vi "Motor_Open.vi"() -> ()   [LabVIEW 2016]
uses:
  <vilib>/Rock Robotics/WPI/SafetyOutput/WPI_SafetyOutputConfigMenu.ctl
  <vilib>/Rock Robotics/WPI/ThirdParty/CanMotor/TalonSRX/WPI_CANTalonSRX_APIControlMode.ctl
  ArgosLib/Drive/MotorControl/TypeDefs/RobotDriveMotorSelectorEnum.ctl
  <vilib>/Rock Robotics/WPI/ThirdParty/CanMotor/TalonSRX/WPI_CANTalonSRX_APIFeedbackSelect.ctl
  Global_Var-RefNum/Global_Var_Drive.vi
  ArgosLib/Drive/MotorControl/RobotDriveOpen6MotorWithTalonSRX.vi
  ArgosLib/ArgosLib.lvlib
panel:
  in  "Left Motor 1 Inverted_P":bool
  in  "Left Motor 2 Inverted_P":bool
  in  "Right Motor 1 Inverted_P":bool
  in  "Right Motor 2 Inverted_P":bool
  in  "Left Motor 1 Inverted":bool
  in  "Left Motor 2 Inverted":bool
  in  "Right Motor 1 Inverted":bool
  in  "Right Motor 2 Inverted":bool
  # "Practice"
  # "Competition"
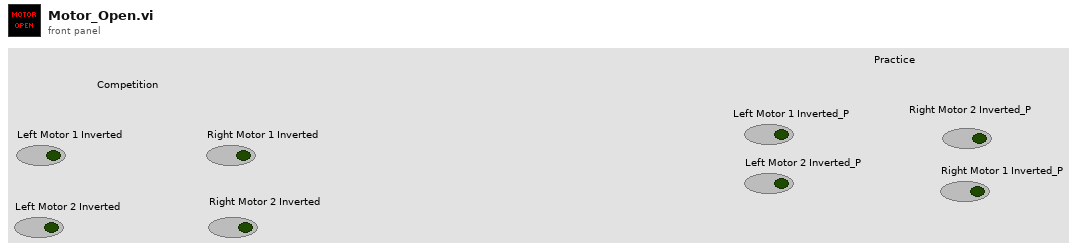
[diagram p1: front panel]
types:
  T1 = typedef "WPI_SafetyOutputConfigMenu.ctl" = enum16{"Enable", "Disable"}
  T2 = typedef "WPI_CANTalonSRX_APIControlMode.ctl" = enum8{"Percent VBus", "Speed", "Position", "Slave", "Unchanged / Invalid", "Voltage Compensation", "Current", "Motion Profile", "Motion Magic"}
  T3 = typedef "ArgosLib.lvlib/RobotDriveMotorSelectorEnum.ctl" = enum16{"Left Motor 1", "Right Motor 1", "Left Motor 2", "Right Motor 2", "Left Motor 3", "Right Motor 3"}
  T4 = typedef "WPI_RobotDriveDevRef.ctl" = cluster{"DevStatus":errorcluster, "Motors[]":T5[], "Square Inputs":bool, "Max Output":dbl}
  T5 = typedef "WPI_MotorControlDeviceRef.ctl" = cluster{"DeviceStatus":errorcluster, "Type":T6, "PWM":cluster{"PWM Channel":T7, "DeadBand":T8}, "CAN":cluster{"Device Number":u8, "SetOutput VI Ref":variant, "GetOutput VI Ref":variant, "Enable VI Ref":variant, "Disable VI Ref":variant, "Data":variant}, "Invert":bool}
  T6 = typedef "WPI_MotorControlType.ctl" = enum16{"PWM", "CAN"}
  T7 = typedef "FPGA_DIOPWMChannel.ctl" = enum8{"PWM 0", "PWM 1", "PWM 2", "PWM 3", "PWM 4", "PWM 5", "PWM 6", "PWM 7", "PWM 8", "PWM 9", "PWM MXP 0", "PWM MXP 1", "PWM MXP 2", "PWM MXP 3", "PWM MXP 4", "PWM MXP 5", "PWM MXP 6", "PWM MXP 7", "PWM MXP 8", "PWM MXP 9", "Invalid"}
  T8 = typedef "WPI_PWMDeadband.ctl" = cluster{"Name":string, "maxPositivePwm":i32, "minPositivePwm":i32, "centerPwm":i32, "maxNegativePwm":i32, "minNegativePwm":i32, "angularRange":u16}
  T9 = typedef "WPI_CANTalonSRX_APIFeedbackSelect.ctl" = enum16{"Digital Quadrature Encoder", "Analog Potentiometer", "Analog Encoder", "Count on Quad-A (Rising-Edge)", "Count on Quad-A (Falling-Edge)", "CTR Magnetic Enc (Absolute)", "CTR Magnetic Enc (Relative)", "Pulse Width"}
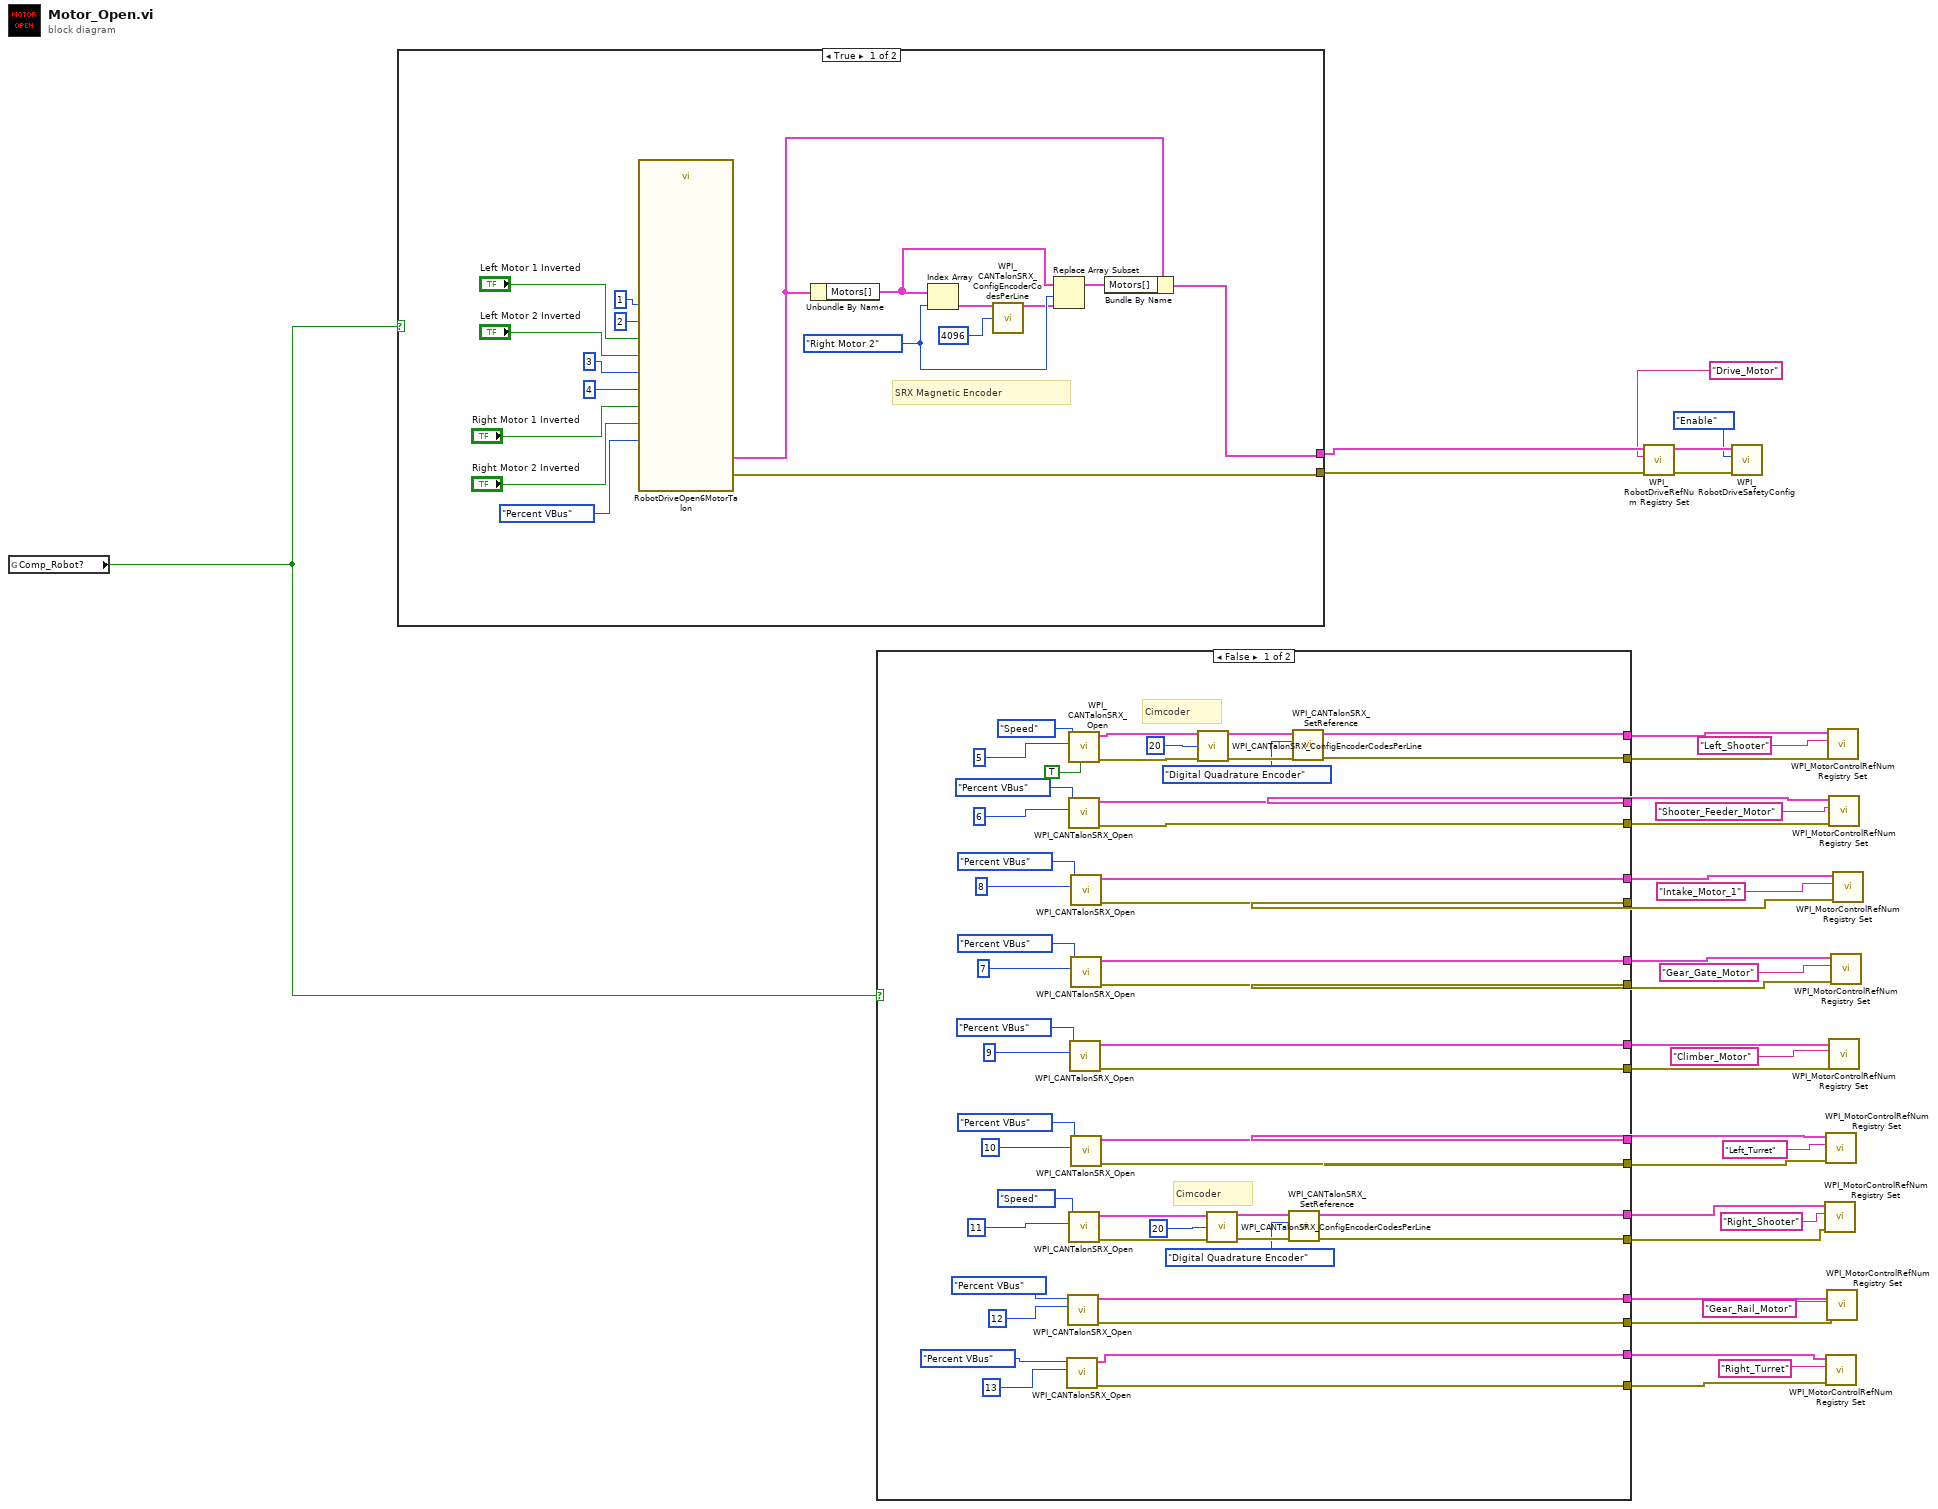
[diagram p0: block diagram]
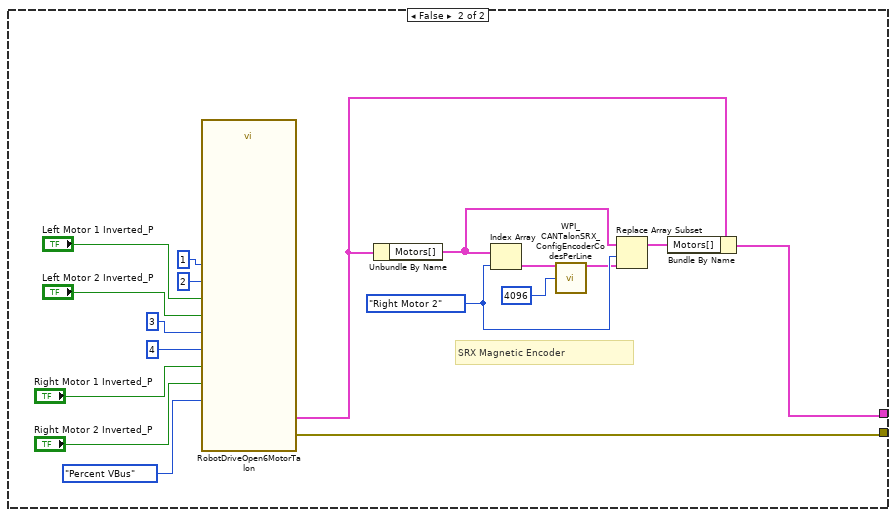
[diagram p2: hidden frame]
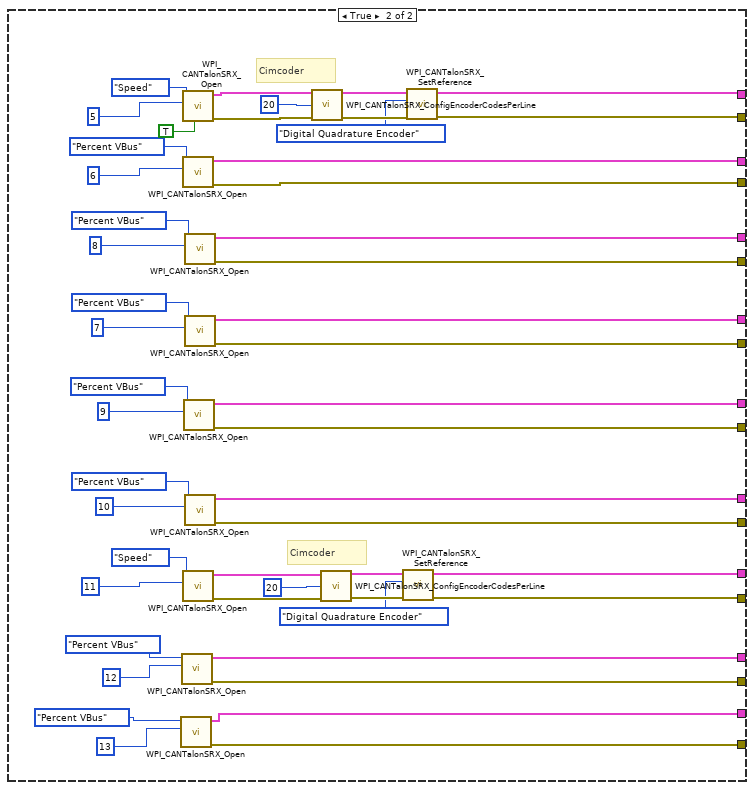
[diagram p3: hidden frame]
diagram:
  n1 = global read "Global_Var_Drive.vi" "Comp_Robot?"() -> (w4:bool)
  n2 = case shown="True" w4 {
    tunnel: [w43 w61] -> w34
    tunnel: [w35 w53] -> w33
    frame True {
      w39 = RobotDriveMotorSelectorEnum."Right Motor 2" ("Motor Selector Enum")
      # "SRX Magnetic Encoder"
      n3 = call-poly "RobotDriveOpen6MotorTalon.vi"("Left Motor 1"=u8 1, "Left Motor 2"=u8 2, "Right Motor 1"=u8 3, "Right Motor 2"=u8 4, "Left Motor 1 Inverted"="Left Motor 1 Inverted", "Right Motor 1 Inverted"="Right Motor 1 Inverted", "Left Motor 2 Inverted"="Left Motor 2 Inverted", "Right Motor 2 Inverted"="Right Motor 2 Inverted", "Control Mode"=WPI_CANTalonSRX_APIControlMode."Percent VBus") -> ("RobotDriveDevRef"=w36:T4, "error out"=w43:errorcluster)  [unwired: 17 in]
      n4 = Unbundle By Name(w36) -> ("Motors[]"=w40:T5[])
      n5 = Index Array(array=w40, index=w39) -> (element=w42:T5)
      n6 = call <vilib>:"WPI_CANTalonSRX_ConfigEncoderCodesPerLine.vi"("CAN Talon SRX Ref"=w42, "Number Encoder Lines\n(Counts Per Rotation)"=u32 4096 ("Number Encoder Lines\n(Counts Per Rotation)")) -> ("CAN Talon SRX Ref"=w38:T5)  [unwired: 12 in, 1 out]
      n7 = Replace Array Subset(array=w40, new element=w38, index=w39) -> (w37:T5[])
      n8 = Bundle By Name(cluster=w36, "Motors[]"=w37) -> (w35:T4)
    }
    frame False {
      w57 = RobotDriveMotorSelectorEnum."Right Motor 2" ("Motor Selector Enum")
      # "SRX Magnetic Encoder"
      n9 = call-poly "RobotDriveOpen6MotorTalon.vi"("Left Motor 1"=u8 1, "Left Motor 2"=u8 2, "Right Motor 1"=u8 3, "Right Motor 2"=u8 4, "Left Motor 1 Inverted"="Left Motor 1 Inverted_P", "Right Motor 1 Inverted"="Right Motor 1 Inverted_P", "Left Motor 2 Inverted"="Left Motor 2 Inverted_P", "Right Motor 2 Inverted"="Right Motor 2 Inverted_P", "Control Mode"=WPI_CANTalonSRX_APIControlMode."Percent VBus") -> ("RobotDriveDevRef"=w54:T4, "error out"=w61:errorcluster)  [unwired: 17 in]
      n10 = Unbundle By Name(w54) -> ("Motors[]"=w58:T5[])
      n11 = Index Array(array=w58, index=w57) -> (element=w60:T5)
      n12 = call <vilib>:"WPI_CANTalonSRX_ConfigEncoderCodesPerLine.vi"("CAN Talon SRX Ref"=w60, "Number Encoder Lines\n(Counts Per Rotation)"=u32 4096 ("Number Encoder Lines\n(Counts Per Rotation)")) -> ("CAN Talon SRX Ref"=w56:T5)  [unwired: 12 in, 1 out]
      n13 = Replace Array Subset(array=w58, new element=w56, index=w57) -> (w55:T5[])
      n14 = Bundle By Name(cluster=w54, "Motors[]"=w55) -> (w53:T4)
    }
  }
  n15 = case shown="False" w4 {
    tunnel: [w75 w124] -> w22
    tunnel: [w73 w122] -> w21
    tunnel: [w93 w142] -> w20
    tunnel: [w107 w156] -> w19
    tunnel: [w94 w143] -> w18
    tunnel: [w106 w155] -> w17
    tunnel: [w88 w137] -> w16
    tunnel: [w105 w154] -> w15
    tunnel: [w92 w141] -> w14
    tunnel: [w104 w153] -> w13
    tunnel: [w91 w140] -> w12
    tunnel: [w103 w152] -> w11
    tunnel: [w79 w128] -> w10
    tunnel: [w77 w126] -> w9
    tunnel: [w90 w139] -> w7
    tunnel: [w98 w147] -> w6
    tunnel: [w97 w146] -> w3
    tunnel: [w89 w138] -> w1
    frame False {
      # "Cimcoder"
      # "Cimcoder"
      n16 = call <vilib>:"WPI_CANTalonSRX_Open.vi"("Device Number"=u8 13, "Control Mode"=WPI_CANTalonSRX_APIControlMode."Percent VBus") -> ("error out"=w97:errorcluster, "CAN Talon SRX Ref"=w89:T5)  [unwired: 8 in]
      n17 = call <vilib>:"WPI_CANTalonSRX_Open.vi"("Device Number"=u8 12, "Control Mode"=WPI_CANTalonSRX_APIControlMode."Percent VBus") -> ("error out"=w98:errorcluster, "CAN Talon SRX Ref"=w90:T5)  [unwired: 8 in]
      n18 = call <vilib>:"WPI_CANTalonSRX_Open.vi"("Invert"=TRUE, "Device Number"=u8 5, "Control Mode"=WPI_CANTalonSRX_APIControlMode."Speed") -> ("error out"=w81:errorcluster, "CAN Talon SRX Ref"=w87:T5)  [unwired: 7 in]
      n19 = call <vilib>:"WPI_CANTalonSRX_Open.vi"("Device Number"=u8 6, "Control Mode"=WPI_CANTalonSRX_APIControlMode."Percent VBus") -> ("error out"=w107:errorcluster, "CAN Talon SRX Ref"=w93:T5)  [unwired: 8 in]
      n20 = call <vilib>:"WPI_CANTalonSRX_Open.vi"("Device Number"=u8 11, "Control Mode"=WPI_CANTalonSRX_APIControlMode."Speed") -> ("error out"=w80:errorcluster, "CAN Talon SRX Ref"=w84:T5)  [unwired: 8 in]
      n21 = call <vilib>:"WPI_CANTalonSRX_Open.vi"("Device Number"=u8 9, "Control Mode"=WPI_CANTalonSRX_APIControlMode."Percent VBus") -> ("error out"=w104:errorcluster, "CAN Talon SRX Ref"=w92:T5)  [unwired: 8 in]
      n22 = call <vilib>:"WPI_CANTalonSRX_Open.vi"("Device Number"=u8 8, "Control Mode"=WPI_CANTalonSRX_APIControlMode."Percent VBus") -> ("error out"=w106:errorcluster, "CAN Talon SRX Ref"=w94:T5)  [unwired: 8 in]
      n23 = call <vilib>:"WPI_CANTalonSRX_Open.vi"("Device Number"=u8 7, "Control Mode"=WPI_CANTalonSRX_APIControlMode."Percent VBus") -> ("error out"=w105:errorcluster, "CAN Talon SRX Ref"=w88:T5)  [unwired: 8 in]
      n24 = call <vilib>:"WPI_CANTalonSRX_Open.vi"("Device Number"=u8 10, "Control Mode"=WPI_CANTalonSRX_APIControlMode."Percent VBus") -> ("error out"=w103:errorcluster, "CAN Talon SRX Ref"=w91:T5)  [unwired: 8 in]
      n25 = call <vilib>:"WPI_CANTalonSRX_ConfigEncoderCodesPerLine.vi"("CAN Talon SRX Ref"=w87, "Number Encoder Lines\n(Counts Per Rotation)"=u32 20 ("Number Encoder Lines\n(Counts Per Rotation)"), "error in (no error)"=w81) -> ("CAN Talon SRX Ref"=w86:T5, "error out"=w74:errorcluster)  [unwired: 11 in]
      n26 = call <vilib>:"WPI_CANTalonSRX_ConfigEncoderCodesPerLine.vi"("CAN Talon SRX Ref"=w84, "Number Encoder Lines\n(Counts Per Rotation)"=u32 20 ("Number Encoder Lines\n(Counts Per Rotation)"), "error in (no error)"=w80) -> ("CAN Talon SRX Ref"=w83:T5, "error out"=w78:errorcluster)  [unwired: 11 in]
      n27 = call <vilib>:"WPI_CANTalonSRX_SetReference.vi"("error in (no error)"=w78, "Feedback Reference"=WPI_CANTalonSRX_APIFeedbackSelect."Digital Quadrature Encoder", "CAN Talon SRX Ref"=w83) -> ("error out"=w77:errorcluster, "CAN Talon SRX Ref"=w79:T5)  [unwired: 7 in]
      n28 = call <vilib>:"WPI_CANTalonSRX_SetReference.vi"("error in (no error)"=w74, "Feedback Reference"=WPI_CANTalonSRX_APIFeedbackSelect."Digital Quadrature Encoder", "CAN Talon SRX Ref"=w86) -> ("error out"=w73:errorcluster, "CAN Talon SRX Ref"=w75:T5)  [unwired: 7 in]
    }
    frame True {
      # "Cimcoder"
      # "Cimcoder"
      n29 = call <vilib>:"WPI_CANTalonSRX_Open.vi"("Device Number"=u8 13, "Control Mode"=WPI_CANTalonSRX_APIControlMode."Percent VBus") -> ("error out"=w146:errorcluster, "CAN Talon SRX Ref"=w138:T5)  [unwired: 8 in]
      n30 = call <vilib>:"WPI_CANTalonSRX_Open.vi"("Device Number"=u8 12, "Control Mode"=WPI_CANTalonSRX_APIControlMode."Percent VBus") -> ("error out"=w147:errorcluster, "CAN Talon SRX Ref"=w139:T5)  [unwired: 8 in]
      n31 = call <vilib>:"WPI_CANTalonSRX_Open.vi"("Invert"=TRUE, "Device Number"=u8 5, "Control Mode"=WPI_CANTalonSRX_APIControlMode."Speed") -> ("error out"=w130:errorcluster, "CAN Talon SRX Ref"=w136:T5)  [unwired: 7 in]
      n32 = call <vilib>:"WPI_CANTalonSRX_Open.vi"("Device Number"=u8 6, "Control Mode"=WPI_CANTalonSRX_APIControlMode."Percent VBus") -> ("error out"=w156:errorcluster, "CAN Talon SRX Ref"=w142:T5)  [unwired: 8 in]
      n33 = call <vilib>:"WPI_CANTalonSRX_Open.vi"("Device Number"=u8 11, "Control Mode"=WPI_CANTalonSRX_APIControlMode."Speed") -> ("error out"=w129:errorcluster, "CAN Talon SRX Ref"=w133:T5)  [unwired: 8 in]
      n34 = call <vilib>:"WPI_CANTalonSRX_Open.vi"("Device Number"=u8 9, "Control Mode"=WPI_CANTalonSRX_APIControlMode."Percent VBus") -> ("error out"=w153:errorcluster, "CAN Talon SRX Ref"=w141:T5)  [unwired: 8 in]
      n35 = call <vilib>:"WPI_CANTalonSRX_Open.vi"("Device Number"=u8 8, "Control Mode"=WPI_CANTalonSRX_APIControlMode."Percent VBus") -> ("error out"=w155:errorcluster, "CAN Talon SRX Ref"=w143:T5)  [unwired: 8 in]
      n36 = call <vilib>:"WPI_CANTalonSRX_Open.vi"("Device Number"=u8 7, "Control Mode"=WPI_CANTalonSRX_APIControlMode."Percent VBus") -> ("error out"=w154:errorcluster, "CAN Talon SRX Ref"=w137:T5)  [unwired: 8 in]
      n37 = call <vilib>:"WPI_CANTalonSRX_Open.vi"("Device Number"=u8 10, "Control Mode"=WPI_CANTalonSRX_APIControlMode."Percent VBus") -> ("error out"=w152:errorcluster, "CAN Talon SRX Ref"=w140:T5)  [unwired: 8 in]
      n38 = call <vilib>:"WPI_CANTalonSRX_ConfigEncoderCodesPerLine.vi"("CAN Talon SRX Ref"=w136, "Number Encoder Lines\n(Counts Per Rotation)"=u32 20 ("Number Encoder Lines\n(Counts Per Rotation)"), "error in (no error)"=w130) -> ("CAN Talon SRX Ref"=w135:T5, "error out"=w123:errorcluster)  [unwired: 11 in]
      n39 = call <vilib>:"WPI_CANTalonSRX_ConfigEncoderCodesPerLine.vi"("CAN Talon SRX Ref"=w133, "Number Encoder Lines\n(Counts Per Rotation)"=u32 20 ("Number Encoder Lines\n(Counts Per Rotation)"), "error in (no error)"=w129) -> ("CAN Talon SRX Ref"=w132:T5, "error out"=w127:errorcluster)  [unwired: 11 in]
      n40 = call <vilib>:"WPI_CANTalonSRX_SetReference.vi"("error in (no error)"=w127, "Feedback Reference"=WPI_CANTalonSRX_APIFeedbackSelect."Digital Quadrature Encoder", "CAN Talon SRX Ref"=w132) -> ("error out"=w126:errorcluster, "CAN Talon SRX Ref"=w128:T5)  [unwired: 7 in]
      n41 = call <vilib>:"WPI_CANTalonSRX_SetReference.vi"("error in (no error)"=w123, "Feedback Reference"=WPI_CANTalonSRX_APIFeedbackSelect."Digital Quadrature Encoder", "CAN Talon SRX Ref"=w135) -> ("error out"=w122:errorcluster, "CAN Talon SRX Ref"=w124:T5)  [unwired: 7 in]
    }
  }
  n42 = call <vilib>:"WPI_RobotDriveRefNum Registry Set.vi"("error in (no error)"=w34, "refnum name"="Drive_Motor", "RobotDriveDevRef"=w33) -> ("error out"=w31:errorcluster, "RobotDriveDevRef"=w32:T4)  [unwired: 7 in]
  n43 = call <vilib>:"WPI_RobotDriveSafetyConfig.vi"("error in (no error)"=w31, "mode"=WPI_SafetyOutputConfigMenu."Enable", "RobotDriveDevRef"=w32) -> ()  [unwired: 7 in, 2 out]
  n44 = call <vilib>:"WPI_MotorControlRefNum Registry Set.vi"("error in (no error)"=w9, "refnum name"="Right_Shooter", "MotorControlDevRef"=w10) -> ()  [unwired: 7 in, 2 out]
  n45 = call <vilib>:"WPI_MotorControlRefNum Registry Set.vi"("error in (no error)"=w11, "refnum name"="Left_Turret", "MotorControlDevRef"=w12) -> ()  [unwired: 7 in, 2 out]
  n46 = call <vilib>:"WPI_MotorControlRefNum Registry Set.vi"("error in (no error)"=w3, "refnum name"="Right_Turret", "MotorControlDevRef"=w1) -> ()  [unwired: 7 in, 2 out]
  n47 = call <vilib>:"WPI_MotorControlRefNum Registry Set.vi"("error in (no error)"=w6, "refnum name"="Gear_Rail_Motor", "MotorControlDevRef"=w7) -> ()  [unwired: 7 in, 2 out]
  n48 = call <vilib>:"WPI_MotorControlRefNum Registry Set.vi"("error in (no error)"=w21, "refnum name"="Left_Shooter", "MotorControlDevRef"=w22) -> ()  [unwired: 7 in, 2 out]
  n49 = call <vilib>:"WPI_MotorControlRefNum Registry Set.vi"("error in (no error)"=w19, "refnum name"="Shooter_Feeder_Motor", "MotorControlDevRef"=w20) -> ()  [unwired: 7 in, 2 out]
  n50 = call <vilib>:"WPI_MotorControlRefNum Registry Set.vi"("error in (no error)"=w13, "refnum name"="Climber_Motor", "MotorControlDevRef"=w14) -> ()  [unwired: 7 in, 2 out]
  n51 = call <vilib>:"WPI_MotorControlRefNum Registry Set.vi"("error in (no error)"=w15, "refnum name"="Gear_Gate_Motor", "MotorControlDevRef"=w16) -> ()  [unwired: 7 in, 2 out]
  n52 = call <vilib>:"WPI_MotorControlRefNum Registry Set.vi"("error in (no error)"=w17, "refnum name"="Intake_Motor_1", "MotorControlDevRef"=w18) -> ()  [unwired: 7 in, 2 out]
